vi "Selection.vi"   [LabVIEW 2017]
uses:
  <vilib>/myRIO/Instrument Drivers/Onboard IO/DIO/typedefs/DIO Reference.ctl
  <vilib>/myRIO/Common/Instrument Driver Framework/Utilities/typedefs/myRIO Generic Hardware Reference.ctl
  <vilib>/myRIO/Common/Instrument Driver Framework/Utilities/typedefs/Hardware Version Enum.ctl
  <vilib>/myRIO/Common/Instrument Driver Framework/Utilities/typedefs/myRIO v1.0 Reference.ctl
  <vilib>/myRIO/Common/Instrument Driver Framework/Utilities/typedefs/Generic FPGA Reference.ctl
  <vilib>/myRIO/Common/Instrument Driver Framework/myRIO v1.0/DIO/typedefs/DIO Channels List.ctl
  <vilib>/myRIO/Common/Instrument Driver Framework/myRIO v1.0/DIO/typedefs/DIO Channels Enum.ctl
  <vilib>/userdefined/High Color/nirio_resource_hc.ctl
  <vilib>/myRIO/Common/Instrument Driver Framework/Utilities/vis/Is FPGA Ref Available.vi
  <vilib>/myRIO/Common/Instrument Driver Framework/myRIO v1.0/DIO/vis/myRIO v1.1 Open DIO.vi
  <vilib>/myRIO/Instrument Drivers/Onboard IO/DIO/vis/Read.vi
  <vilib>/myRIO/Instrument Drivers/Onboard IO/DIO/vis/Write.vi
  <vilib>/myRIO/Common/Instrument Driver Framework/Utilities/vis/Validate Channels.vi
  <vilib>/myRIO/Common/Instrument Driver Framework/myRIO v1.0/DIO/vis/myRIO v1.0 Reserve DIO.vi
  <vilib>/myRIO/Common/Instrument Driver Framework/myRIO v1.0/Resource Manager/vis/myRIO v1.0 Reserve Channel List.vi
  <vilib>/myRIO/Common/Instrument Driver Framework/myRIO v1.0/DIO/vis/myRIO v1.0 Build MUX Configuration DIO.vi
  <vilib>/myRIO/Common/Instrument Driver Framework/myRIO v1.0/Resource Manager/vis/myRIO v1.0 Reserve Channel.vi
  <vilib>/myRIO/Common/Instrument Driver Framework/myRIO v1.0/Resource Manager/vis/myRIO v1.0 Unreserve Channel.vi
  <vilib>/myRIO/Common/Instrument Driver Framework/myRIO v1.0/Resource Manager/vis/myRIO v1.0 Create Configuration List.vi
  <vilib>/myRIO/Common/Instrument Driver Framework/myRIO v1.0/Resource Manager/vis/myRIO v1.0 Build Mutex Name.vi
  <vilib>/Utility/VariantDataType/GetNumericInfo.vi
  <vilib>/Utility/error.llb/Error Cluster From Error Code.vi
  <vilib>/myRIO/Common/Instrument Driver Framework/myRIO v1.0/myRIO v1.1 Open.vi
  <vilib>/myRIO/Common/Instrument Driver Framework/Utilities/vis/IO Manager.vi
  <vilib>/myRIO/Common/Instrument Driver Framework/Utilities/vis/Configuration Manager.vi
  <vilib>/myRIO/Common/Instrument Driver Framework/myRIO v1.0/Resource Manager/vis/myRIO v1.0 Configure IO.vi
  <vilib>/myRIO/Common/Instrument Driver Framework/myRIO v1.0/myRIO v1.0 Close.vi
  <vilib>/myRIO/Common/Instrument Driver Framework/myRIO v1.0/DIO/vis/myRIO v1.0 Read DIO.vi
  <vilib>/myRIO/Common/Instrument Driver Framework/myRIO v1.0/DIO/vis/myRIO v1.0 Write DIO.vi
  <vilib>/myRIO/Express VI/Onboard Devices/Button/Button Express VI.xnode
  <vilib>/myRIO/Instrument Drivers/Onboard IO/DIO/vis/myRIO DIO Open.xnode
  <vilib>/myRIO/Express VI/Onboard Devices/LED/LED Express VI.xnode
  <vilib>/myRIO/Instrument Drivers/Onboard IO/DIO/DIO.lvlib
types:
  T1 = enum16{"Initialisation", "Prog1", "Prog2", "Prog3"}
  T2 = typedef "DIO.lvlib/DIO Reference.ctl" = cluster{"myRIO Reference":T3, "DIO Channels List":T7}
  T3 = typedef "myRIO Generic Hardware Reference.ctl" = cluster{"myRIO Model":T4, "myRIO Hardware Reference":T5}
  T4 = typedef "Hardware Version Enum.ctl" = enum16{"Unknown", "myRIO-1900", "myRIO-1950", "roboRIO", "NI ELVIS RIO CM"}
  T5 = typedef "myRIO v1.0 Reference.ctl" = cluster{"Generic FPGA Reference":T6, "Allow multiple opens":bool}
  T6 = typedef "Generic FPGA Reference.ctl" = refnum<k20>
  T7 = typedef "DIO Channels List.ctl" = T8[]
  T8 = typedef "DIO Channels Enum.ctl" = enum16{"Not Connected", "C/DIO0", "C/DIO1", "C/DIO2", "C/DIO3", "C/DIO4", "C/DIO5", "C/DIO6", "C/DIO7", "A/DIO0", "A/DIO1", "A/DIO2", "A/DIO3", "A/DIO4", "A/DIO5", "A/DIO6", "A/DIO7", "A/DIO8", "A/DIO9", "A/DIO10", "A/DIO11", "A/DIO12", "A/DIO13", "A/DIO14", "A/DIO15", "B/DIO0", "B/DIO1", "B/DIO2", "B/DIO3", "B/DIO4", "B/DIO5", "B/DIO6", "B/DIO7", "B/DIO8", "B/DIO9", "B/DIO10", "B/DIO11", "B/DIO12", "B/DIO13", "B/DIO14", "B/DIO15", "LED0", "LED1", "LED2", "LED3", "Button0", "DIO/DIO0", "DIO/DIO1", "DIO/DIO2", "DIO/DIO3", "DIO/DIO4", "DIO/DIO5", "DIO/DIO6", "DIO/DIO7", "DIO/DIO8", "DIO/DIO9", "SPI/CS0", "SPI/CS1", "SPI/CS2", "SPI/CS3", "LED RADIO (Green)", "LED RADIO (Red)", "LED COMM (Green)", "LED COMM (Red)", "LED MODE (Green)", "LED MODE (Red)"}
  T9 = typedef "nirio_resource_hc.ctl" = tag
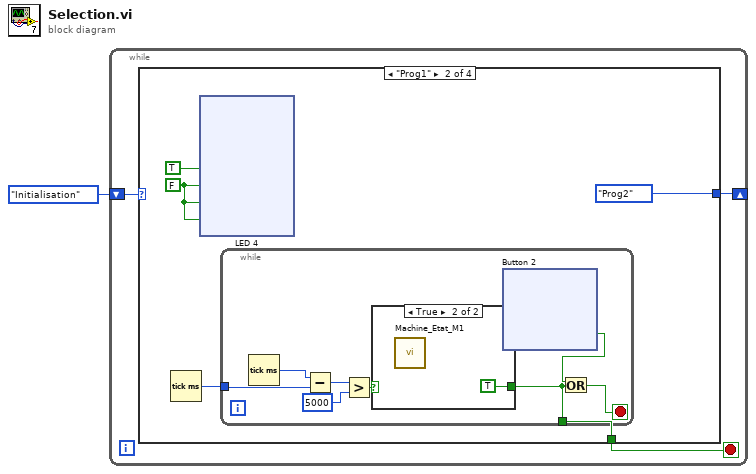
[diagram p0: block diagram]
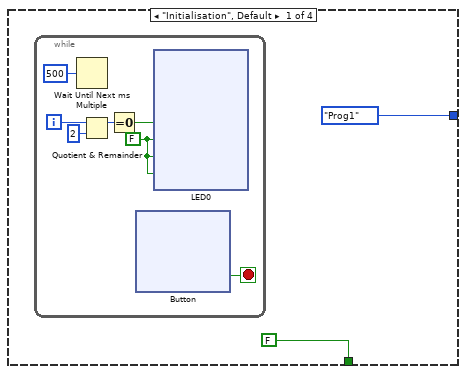
[diagram p2: hidden frame]
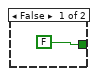
[diagram p3: hidden frame]
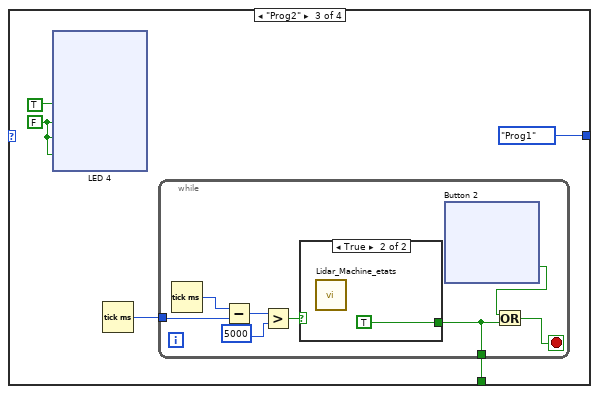
[diagram p4: hidden frame]
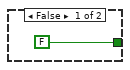
[diagram p5: hidden frame]
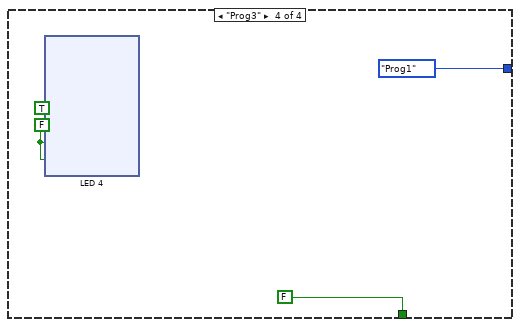
[diagram p6: hidden frame]
diagram:
  n1 = while {
    shift-right: [w3] -> _
    shift-left: T1."Initialisation" -> [w4]
    stop <- w2 stop-if-true
    n2 = case shown="\"Prog1\"" w4 {
      tunnel: [T1."Prog1" T1."Prog2" T1."Prog1" T1."Prog1"] -> w3
      tunnel: [FALSE w87 w175 FALSE] -> w2
      frame "Initialisation", Default {
        n3 = while {
          i -> [w11]
          stop <- w13 stop-if-true
          w7 = FALSE ("LED1")
          n4 = Wait Until Next ms Multiple(millisecond multiple=u32 500 ("n millisecondes")) -> ()  [unwired: 1 out]
          n5 = Quotient & Remainder(x=w11, y=2) -> (x-y*floor(x/y)=w9:i32)  [unwired: 1 out]
          n6 = Equal To 0?(x=w9) -> (x = 0?=w8:bool)
          n7 = xnode "Button"() -> ("Value"=w13:bool)  [unwired: 1 in, 1 out]
          n8 = xnode "LED0"("LED0"=w8, "LED1"=w7, "LED2"=w7, "LED3"=w7) -> ()  [unwired: 1 in, 1 out]
        }
      }
      frame "Prog1" {
        w89 = FALSE ("LED1")
        n9 = Tick Count (ms)() -> (millisecond timer value=w88:u32)
        n10 = xnode "LED 4"("LED1"=TRUE ("LED0"), "LED0"=w89, "LED2"=w89, "LED3"=w89) -> ()  [unwired: 1 in, 1 out]
        n11 = while {
          tunnel: w88 -> [w98]
          tunnel: [w92] -> w87
          stop <- w94 stop-if-true
          n12 = Tick Count (ms)() -> (millisecond timer value=w99:u32)
          n13 = Subtract(x=w99, y=w98) -> (x-y=w97:u32)
          n14 = Greater?(x=w97, y=u32 5000) -> (0:w95:bool)
          n15 = case shown="True" w95 {
            tunnel: [FALSE TRUE] -> w92
            frame False {
            }
            frame True {
              n16 = call "Machine_Etat_M1.vi"() -> ()  [unwired: 12 in]
            }
          }
          n17 = xnode "Button 2"() -> ("Value"=w93:bool)  [unwired: 1 in, 1 out]
          n18 = Or(x=w93, y=w92) -> (x .or. y?=w94:bool)
        }
      }
      frame "Prog2" {
        w177 = FALSE ("LED1")
        n19 = xnode "LED 4"("LED2"=TRUE ("LED0"), "LED0"=w177, "LED1"=w177, "LED3"=w177) -> ()  [unwired: 1 in, 1 out]
        n20 = Tick Count (ms)() -> (millisecond timer value=w176:u32)
        n21 = while {
          tunnel: w176 -> [w186]
          tunnel: [w180] -> w175
          stop <- w181 stop-if-true
          n22 = Tick Count (ms)() -> (millisecond timer value=w187:u32)
          n23 = Subtract(x=w187, y=w186) -> (x-y=w185:u32)
          n24 = Greater?(x=w185, y=u32 5000) -> (0:w183:bool)
          n25 = case shown="True" w183 {
            tunnel: [FALSE TRUE] -> w180
            frame False {
            }
            frame True {
              n26 = call "Lidar_Machine_etats.vi"() -> ()  [unwired: 12 in]
            }
          }
          n27 = xnode "Button 2"() -> ("Value"=w182:bool)  [unwired: 1 in, 1 out]
          n28 = Or(x=w182, y=w180) -> (x .or. y?=w181:bool)
        }
      }
      frame "Prog3" {
        w265 = FALSE ("LED1")
        n29 = xnode "LED 4"("LED3"=TRUE ("LED0"), "LED0"=w265, "LED1"=w265, "LED2"=w265) -> ()  [unwired: 1 in, 1 out]
      }
    }
  }
